vi "GQS Probe.vi"(0 "value":dbl, 11 "error in":errorcluster) -> (4 "elements":dbl[](array[numeric]), 15 "error out":errorcluster)   [LabVIEW 2026]
doc: "Probe: Get Queue Status returns the elements of a double queue."
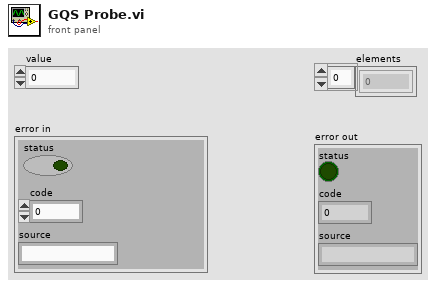
[diagram p1: front panel]
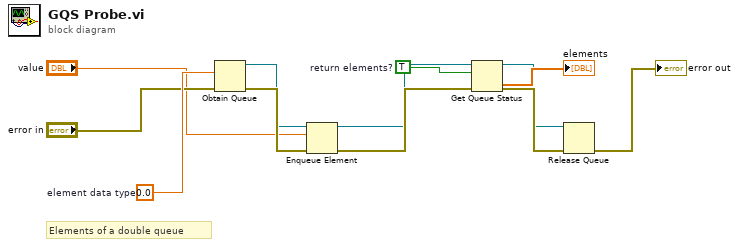
[diagram p0: block diagram]
diagram:
  w4 = TRUE  # return elements?
  w3 = 0.0  # element data type
  # "Elements of a double queue"
  n1 = Obtain Queue(element data type=w3, error in (no error)="error in") -> (queue out=w5:refnum<queue>, error out=w6:errorcluster)  [unwired: 3 in, 1 out]
  n2 = Enqueue Element(queue=w5, element="value", error in (no error)=w6) -> (queue out=w7:refnum<queue>, error out=w8:errorcluster)  [unwired: 1 in, 1 out]
  n3 = Get Queue Status(queue=w7, return elements? (F)=w4, error in (no error)=w8) -> (queue out=w9:refnum<queue>, error out=w11:errorcluster, elements=→"elements":dbl[])  [unwired: 5 out]
  n4 = Release Queue(queue=w9, error in (no error)=w11) -> (error out=→"error out":errorcluster)  [unwired: 1 in, 2 out]
